vi "test unicode import.vi"() -> ()   [LabVIEW 2019, in "Language Editor.lvlib"]
uses:
  Language Editor.lvlib
panel:
  out "Array":string[](array[string])
  out "text":string
  out "unsigned byte array 3":u8[](array[numeric]) format="%.0x"
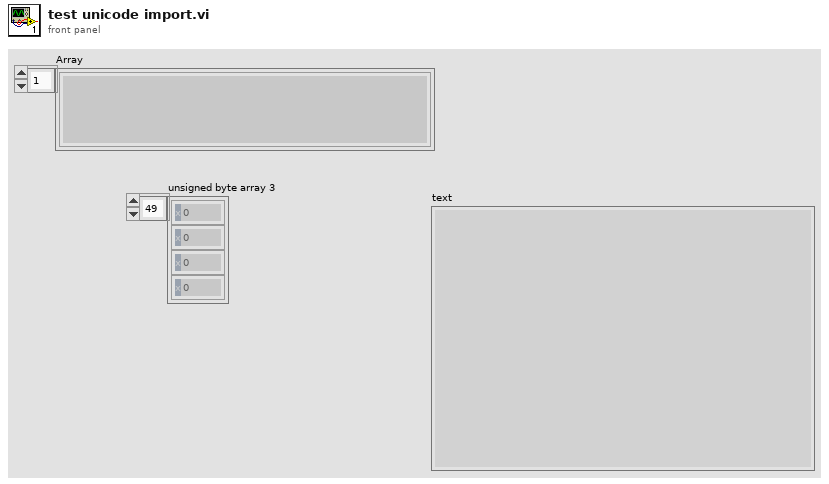
[diagram p1: front panel]
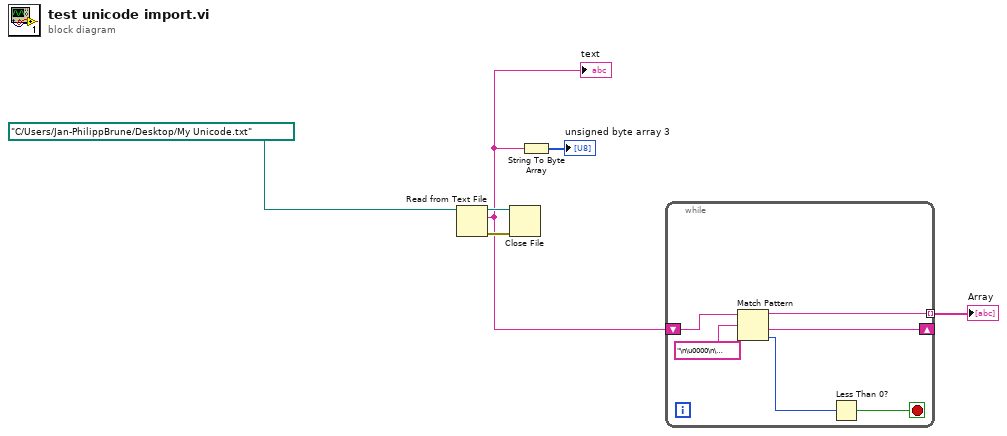
[diagram p0: block diagram]
diagram:
  n1 = Read from Text File(file (use dialog)=path "C:/Users/Jan-PhilippBrune/Desktop/My Unicode.txt") -> (refnum out=w5:refnum<file>, text=w2:string, error out=w6:errorcluster)  [unwired: 3 in, 1 out]
  "text" <- w2
  n2 = Close File(refnum=w5, error in=w6) -> ()  [unwired: 2 out]
  n3 = String To Byte Array(string=w2) -> (unsigned byte array=→"unsigned byte array 3":u8[])
  n4 = while {
    tunnel: [w8] -> w1 mode=indexing
    shift-right: [w7] -> _
    shift-left: w2 -> [w12]
    stop <- w10 stop-if-true
    n5 = Match Pattern(string=w12, regular expression="\n\u0000\n\u0000") -> (before substring=w8:string, after substring=w7:string, offset past match=w11:i32)  [unwired: 1 in, 1 out]
    n6 = Less Than 0?(x=w11) -> (x < 0?=w10:bool)
  }
  "Array" <- w1
